vi "set Average Mode - OBW CHP.vi"(8 "error in (no error)":errorcluster, 10 "Average Mode":enum16{"Exponential", "Repeat"}(ring), 11 "Keysight 9020A in":refnum<class "Keysight 9020A.lvclass">) -> (0 "error out":errorcluster, 3 "Keysight 9020A out":refnum<class "Keysight 9020A.lvclass">)   [LabVIEW 2023, in "Spectrum Analyzer.lvlib" / "Keysight 9020A.lvclass"]
uses:
  Keysight 9020A.lvclass
  Keysight 9020A.lvclass/Keysight 9020A.ctl
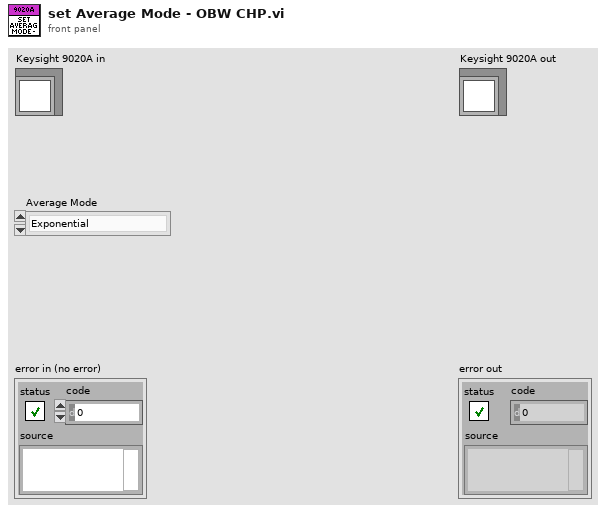
[diagram p1: front panel]
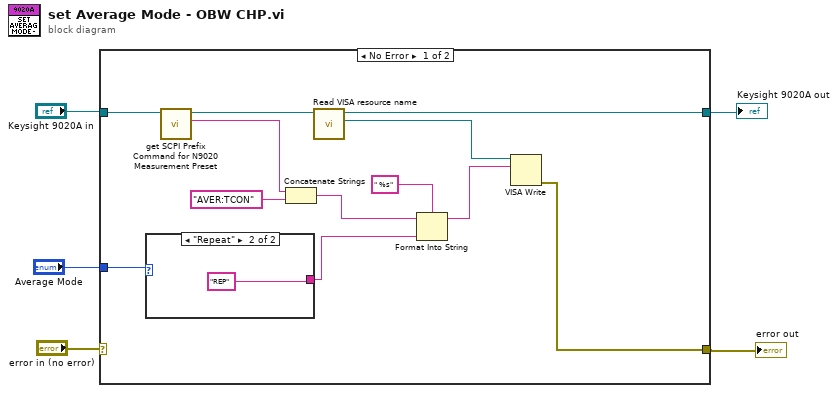
[diagram p0: block diagram]
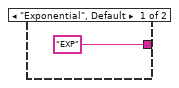
[diagram p2: hidden frame]
diagram:
  n1 = case shown="No Error" "error in (no error)" {
    selector: "error in (no error)" -> [_ w20]
    tunnel: "Keysight 9020A in" -> [w12 w21]
    tunnel: [w17 w21] -> w4
    tunnel: [w13 w20] -> w2
    tunnel: "Average Mode" -> [w7 _]
    frame No Error {
      n2 = case shown="\"Repeat\"" w7 {
        tunnel: ["EXP" "REP"] -> w6
        frame "Exponential", Default {
        }
        frame "Repeat" {
        }
      }
      n3 = call "get SCPI Prefix Command for N9020 Measurement Preset.vi"("Keysight 9020A in"=w12) -> ("SCPI Prefix Command"=w10:string, "Keysight 9020A out"=w9:refnum<class "Keysight 9020A.lvclass">)  [unwired: 8 in, 1 out]
      n4 = Concatenate Strings(w10, "AVER:TCON") -> (w8:string)
      n5 = call "Read VISA resource name.vi"("Keysight 9020A in"=w9) -> ("VISA resource name"=w15:refnum<visa-resource-name>, "Keysight 9020A out"=w17:refnum<class "Keysight 9020A.lvclass">)  [unwired: 8 in, 1 out]
      n6 = Format Into String(format string=" %s", initial string=w8, w6) -> (resulting string=w14:string)  [unwired: 1 in, 1 out]
      n7 = VISA Write(VISA resource name=w15, write buffer=w14) -> (error out=w13:errorcluster)  [unwired: 1 in, 2 out]
    }
    frame Error {
    }
  }
  "error out" <- w2
  "Keysight 9020A out" <- w4
